vi "布尔文本写入.vi"(4 "error in (no error)":errorcluster caption="错误输入（无错误）", 5 "Value":string caption="值", 6 "Container State":T3 caption="容器状态", 7 "Display State In":T1 caption="显示状态输入") -> (0 "error out":errorcluster caption="错误输出", 3 "Display State Out":T1 caption="显示状态输出")   [LabVIEW 2025, in "XButton.lvlib" / "button3.xctl"]
uses:
  button3.xctl
  <vilib>/_xctls/Container State.ctl
  helper loop Events.ctl
  move event.ctl
  <vilib>/_xctls/XControlSupport.lvlib
panel:
  # "将以下值显示控件替换为所需类型的显示控件。\n不要从连线板中删除该显示控件或其它显示控件。\n不要更改连线板模式。\n值显示控件应始终位于连线板输出端自顶部起第三个接线端。"
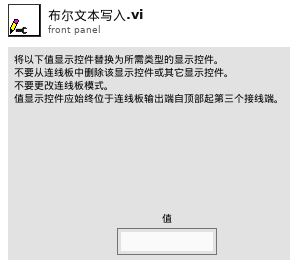
[diagram p1: front panel]
types:
  T1 = typedef "XButton.lvlib/button3.xctl/状态.ctl" = cluster{"Numeric":dbl, "调用方窗格颜色":u32, "按钮颜色":u32, "helper loop data":T2, "布尔文本":string, "字体颜色":u32, "字号":u32, "动效风格":enum16{"风格一", "风格二", "风格三", "风格四"}, "已隐藏不需要遮罩层":bool, "已初始化遮罩层位置":bool}
  T2 = typedef "XButton.lvlib/button3.xctl/helper loop Events.ctl" = cluster{"停止用户事件":refnum<user-event>, "修饰1move用户事件输出":refnum<user-event>, "修饰2move用户事件输出":refnum<user-event>}
  T3 = typedef "XControlSupport.lvlib/Container State.ctl" = cluster{"Indicator?":bool, "Run Mode?":bool, " Refnum":refnum<vi>}
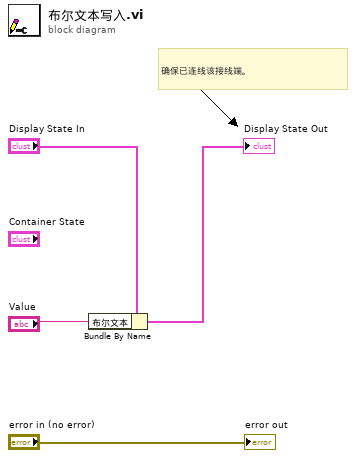
[diagram p0: block diagram]
diagram:
  # "确保已连线该接线端。"
  n1 = Bundle By Name(cluster="Display State In", "布尔文本"="Value") -> (→"Display State Out":T1)
  "error out" <- "error in (no error)"
